vi "Get VI library name.vi"(8 "error in (no error)":errorcluster, 10 "App File Path":path, 11 "VIs":path[](array[path])) -> (0 "error out":errorcluster, 3 "Library or Error String":string[](array[string]))   [LabVIEW 2019, in "Language Editor.lvlib"]
doc: "- - -\nCopyright (c) 2026, Merecs Engineering GmbH"
uses:
  Language Editor.lvlib
panel:
  # "Connector Pane"
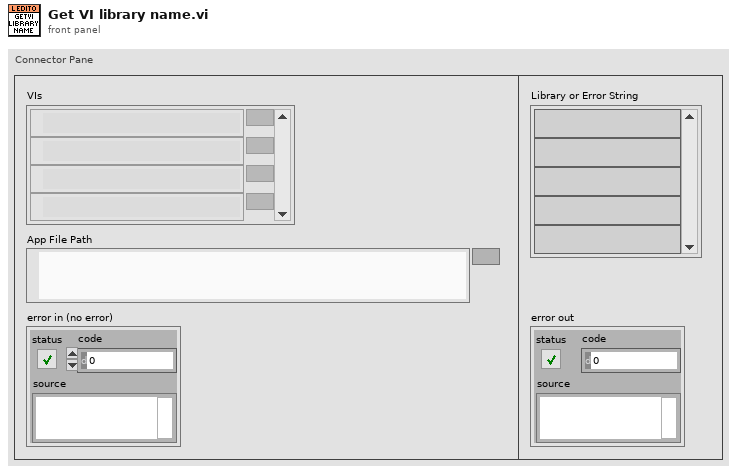
[diagram p1: front panel]
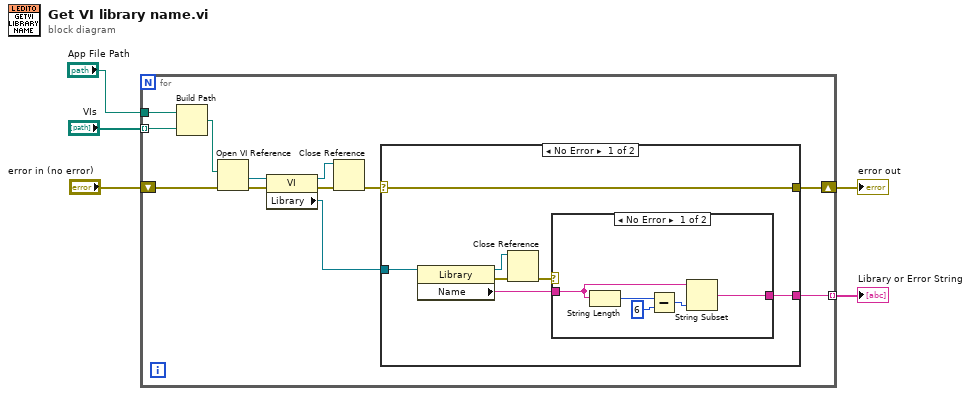
[diagram p0: block diagram]
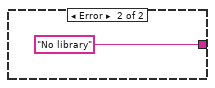
[diagram p2: hidden frame]
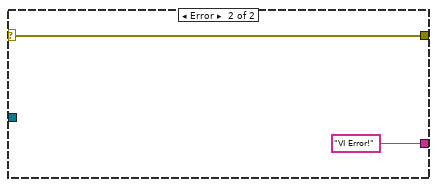
[diagram p3: hidden frame]
diagram:
  n1 = for {
    tunnel: [w16] -> w5 mode=indexing
    tunnel: "VIs" -> [w8] mode=indexing
    shift-right: [w9] -> w3
    shift-left: "error in (no error)" -> [w10]
    tunnel: "App File Path" -> [w6]
    n2 = Build Path(base path=w6, name or relative path=w8) -> (appended path=w7:path)
    n3 = Open VI Reference(vi path=w7, error in (no error)=w10) -> (vi reference=w15:refnum<vi>, error out=w14:errorcluster)  [unwired: 4 in]
    n4 = property class="VI"(reference=w15, error in=w14) -> (reference out=w11:refnum<vi>, error out=w13:errorcluster, "Library"=w17:refnum<vi>)
    n5 = Close Reference(reference=w11, error in (no error)=w13) -> (error out=w12:errorcluster)
    n6 = case shown="No Error" w12 {
      selector: w12 -> [w20 w32]
      tunnel: w17 -> [w24 _]
      tunnel: [w21 "VI Error!" ("Name")] -> w16
      tunnel: [w20 w32] -> w9
      frame No Error {
        n7 = property class="Library"(reference=w24) -> (reference out=w18:refnum<vi>, error out=w23:errorcluster, "Name"=w22:string)  [unwired: 1 in]
        n8 = Close Reference(reference=w18, error in (no error)=w23) -> (error out=w19:errorcluster)
        n9 = case shown="No Error" w19 {
          tunnel: w22 -> [w29 _]
          tunnel: [w25 "No library" ("Name")] -> w21
          frame No Error {
            n10 = String Length(string=w29) -> (length=w28:i32)
            n11 = Subtract(x=w28, y=6) -> (x-y=w26:i32)
            n12 = String Subset(string=w29, length (rest)=w26) -> (substring=w25:string)  [unwired: 1 in]
          }
          frame Error {
          }
        }
      }
      frame Error {
      }
    }
  }
  "Library or Error String" <- w5
  "error out" <- w3
